vi "String to Path.vi"(1 "String":string) -> (0 "Path":path)   [LabVIEW 2017, in "CSM Shared.lvlib"]
uses:
  CSM Shared.lvlib
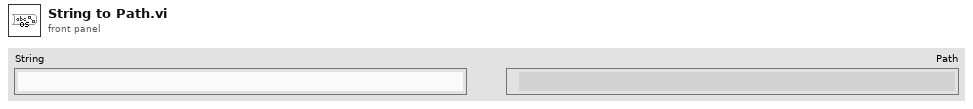
[diagram p1: front panel]
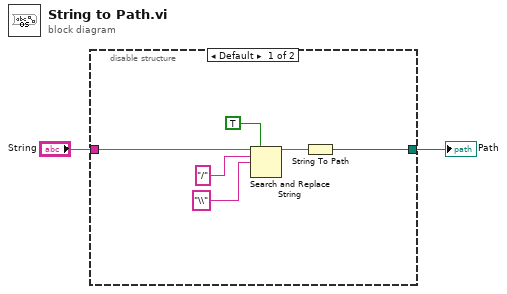
[diagram p0: block diagram]
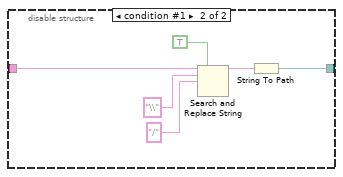
[diagram p2: hidden frame]
diagram:
  n1 = disable-structure shown="Default" {
    disable-tunnel: [w8 w9] -> w2
    disable-tunnel: "String" -> [w3 w14]
    frame condition #0 (active) {
      n2 = Search and Replace String(replace all?=TRUE ("replace all? (F)"), input string=w3, search string="/" ("regular expression"), replace string="\\" ("regular expression")) -> (result string=w6:string)  [unwired: 4 in, 3 out]
      n3 = String To Path(string=w6) -> (path=w8:path)
    }
    frame condition #1 {
      n4 = Search and Replace String(replace all?=TRUE ("replace all? (F)"), input string=w14, search string="\\" ("regular expression"), replace string="/" ("regular expression")) -> (result string=w10:string)  [unwired: 4 in, 3 out]
      n5 = String To Path(string=w10) -> (path=w9:path)
    }
  }
  "Path" <- w2
